vi "UAPublishStructure.vi"(8 "error in (no error)":errorcluster, 10 "OPC UA server refnum in":refnum<k21>, 11 "Server config info":T1) -> (0 "error out":errorcluster, 2 "OPC UA server refnum out":refnum<k21>, 3 "Server config info (dup)":T1)   [LabVIEW 2014, in "OPCUA XML(dev).lvlib"]
uses:
  OPCUA XML(dev).lvlib
  DEF-Server Config Data.ctl
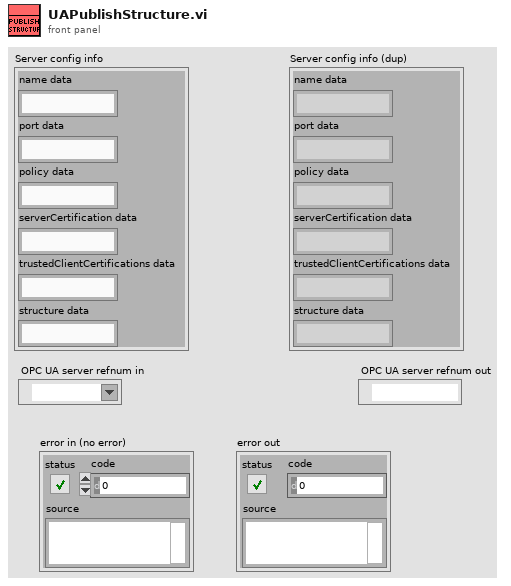
[diagram p1: front panel]
types:
  T1 = typedef "OPCUA XML(dev).lvlib/DEF-Server Config Data.ctl" = cluster{"name data":string, "port data":string, "policy data":string, "serverCertification data":string, "trustedClientCertifications data":string, "structure data":string}
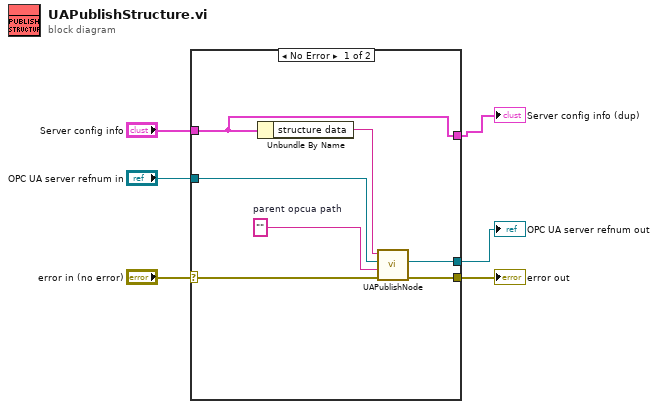
[diagram p0: block diagram]
diagram:
  n1 = case shown="No Error" "error in (no error)" {
    selector: "error in (no error)" -> [w8 w16]
    tunnel: "Server config info" -> [w7 w14]
    tunnel: "OPC UA server refnum in" -> [w11 w15]
    tunnel: [w10 w16] -> w5
    tunnel: [w9 w15] -> w4
    tunnel: [w7 w14] -> w1
    frame No Error {
      w12 = ""  # parent opcua path
      n2 = Unbundle By Name(w7) -> ("structure data"=w13:string)
      n3 = call "UAPublishNode.vi"("error in (no error)"=w8, "parent opcua path"=w12, "OPC UA server refnum in"=w11, "content"=w13) -> ("error out"=w10:errorcluster, "OPC UA server refnum out"=w9:refnum<k21>)  [unwired: 6 in]
    }
    frame Error {
    }
  }
  "error out" <- w5
  "Server config info (dup)" <- w1
  "OPC UA server refnum out" <- w4
